vi "Type Definition Template Name--constant.vi"() -> (3 "Type Definition Template Name":string)   [LabVIEW 2026]
doc: "This constant defines the name of the type definition tempalte."
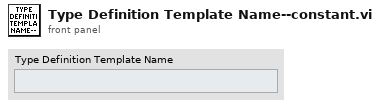
[diagram p1: front panel]
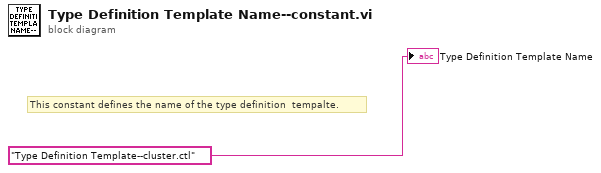
[diagram p0: block diagram]
diagram:
  # "This constant defines the name of the type definition  tempalte."
  "Type Definition Template Name" <- "Type Definition Template--cluster.ctl"
